vi "[ex ce] Curve Length.vi"() -> ()   [LabVIEW 2021]
doc: "CE-Math example.\n\n::: CalcExpress Toolkit :::\nCopyright (c) 2000-2026 Konstantin Shifershteyn. All rights reserved."
uses:
  ce exmpl - 1D difference info.ctl
  <vilib>/gmath/NI_Gmath.lvlib
panel:
  out "max relative difference":T1={"index"=-1, "absolute difference"=0.0, "relative difference, %"=0.0} {"relative difference, %" format="%#.6g"; "absolute difference" format="%#.6g"}
  out "max absolute difference":T1={"index"=-1, "absolute difference"=0.0, "relative difference, %"=0.0} {"relative difference, %" format="%#.6g"; "absolute difference" format="%#.6g"}
  in  "formula info":cluster{"formula":string, "x-variable":string}={"formula"="sinc(x)+sin(2*x)+sin(3*x)+sin(2*x*x)", "x-variable"="x"}
  in  "end":dbl=4.0 format="%.2f"
  in  "start":dbl format="%.2f"
  out "speed ratio":dbl format="%.3f"
  out "GM ticks":u32 caption="ms"
  out "CE ticks":u32 caption="ms"
  out "CE Graph":cluster{"x":dbl[], "f(x)":dbl[]}[](graph) caption="CalcExpress"
  out "GM Graph":cluster{"x":dbl[], "f(x)":dbl[]}[](graph) caption="G Math"
  # "NOTE    CalcExpress uses (^) operator to perform bitwise-XOR operation but not exponentiation operation.\nYou have to use double-asterisk (**) operator to compute an exponent in a CalcExpress expression. For sample, x**y ."
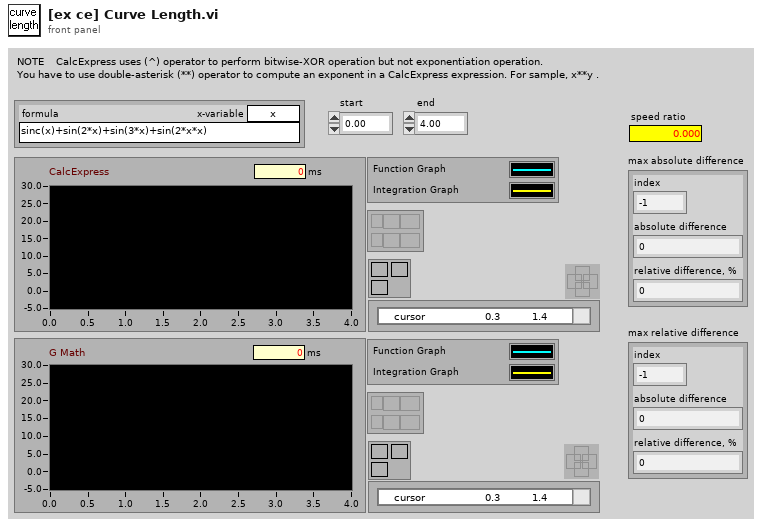
[diagram p1: front panel]
types:
  T1 = typedef "ce exmpl - 1D difference info.ctl" = cluster{"index":i32, "absolute difference":dbl, "relative difference, %":dbl}
  T2 = cluster{"X Values":dbl[], "Curve Length":dbl[]}[]
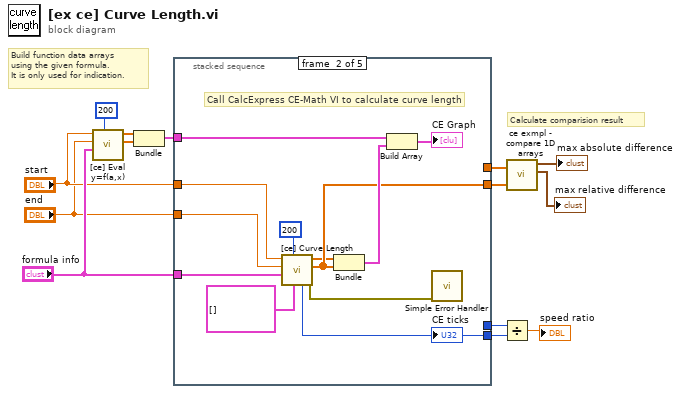
[diagram p0: block diagram]
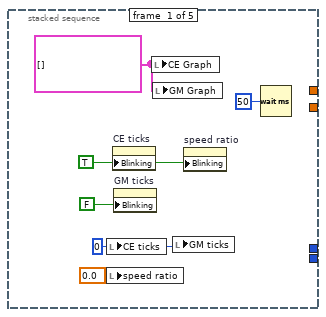
[diagram p2: hidden frame]
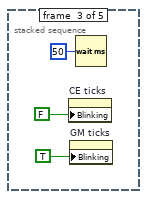
[diagram p3: hidden frame]
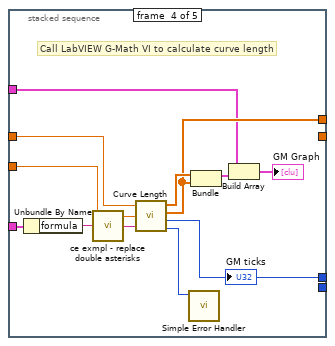
[diagram p4: hidden frame]
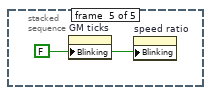
[diagram p5: hidden frame]
diagram:
  # "Calculate comparision result"
  # "Build function data arrays\nusing the given formula.\nIt is only used for indication."
  n1 = call "[ce] Eval y=f(a,x).vi"("# points"=u32 200, "formula info"="formula info", "end"="end", "start"="start") -> ("Y Values"=w6:dbl[], "X Values"=w7:dbl[])  [unwired: 4 in, 2 out]
  n2 = Bundle("X Values"=w7, "Y Values"=w6) -> (w5:cluster{"X Values":dbl[], "Y Values":dbl[]})  [unwired: 1 in]
  n3 = stacked-sequence {
    tunnel: "start" -> [_ w24 _ w43 _]
    tunnel: "end" -> [_ w23 _ w44 _]
    tunnel: "formula info" -> [_ w25 _ w42 _]
    tunnel: [_ w31 _ _ _] -> w14
    tunnel: [_ _ _ w45 _] -> w12
    tunnel: [_ _ _ w37 _] -> w11
    tunnel: [_ w28 _ _ _] -> w10
    tunnel: w5 -> [_ w21 _ w36 _]
    frame #0 {
      w15 = cluster{"x":dbl[], "f(x)":dbl[]}[] [] ("CE Graph")
      w17 = u32 0 ("CE ticks")
      w19 = TRUE ("Write Attribute")
      n4 = local write "CE ticks"(w17) -> ()
      n5 = local write "speed ratio"(0.0 ("speed ratio")) -> ()
      n6 = property on="CE ticks" class="DigNum (strict)"("Blinking"=w19) -> ()  [unwired: 2 in, 2 out]
      n7 = property on="GM ticks" class="DigNum (strict)"("Blinking"=FALSE ("Write Attribute")) -> ()  [unwired: 2 in, 2 out]
      n8 = local write "CE Graph"(w15) -> ()
      n9 = local write "GM Graph"(w15) -> ()
      n10 = local write "GM ticks"(w17) -> ()
      n11 = property on="speed ratio" class="DigNum (strict)"("Blinking"=w19) -> ()  [unwired: 2 in, 2 out]
      n12 = Wait (ms)(milliseconds to wait=u32 50) -> ()  [unwired: 1 out]
    }
    frame #1 {
      # "Call CalcExpress CE-Math VI to calculate curve length"
      n13 = call "[ce] Curve Length.vi"("parameters"=cluster{"name":string, "value":dbl}[] [] ("additional parameters"), "# points"=u32 200, "formula info"=w25, "end"=w23, "start"=w24) -> ("error out"=w32:errorcluster, "ticks"=w31:u32, "Curve Length"=w28:dbl[], "X Values"=w27:dbl[])  [unwired: 3 in]
      "CE ticks" <- w31
      n14 = Bundle("X Values"=w27, "Curve Length"=w28) -> (w30:cluster{"X Values":dbl[], "Curve Length":dbl[]})  [unwired: 1 in]
      n15 = Build Array(w21, w30) -> (→"CE Graph":T2)
      n16 = call <vilib>:"Simple Error Handler.vi"("error in (no error)"=w32) -> ()  [unwired: 4 in, 5 out]
    }
    frame #2 {
      n17 = property on="CE ticks" class="DigNum (strict)"("Blinking"=FALSE ("Write Attribute")) -> ()  [unwired: 2 in, 2 out]
      n18 = property on="GM ticks" class="DigNum (strict)"("Blinking"=TRUE ("Write Attribute")) -> ()  [unwired: 2 in, 2 out]
      n19 = Wait (ms)(milliseconds to wait=u32 50) -> ()  [unwired: 1 out]
    }
    frame #3 {
      # "Call LabVIEW G-Math VI to calculate curve length"
      n20 = Unbundle By Name(w42) -> ("formula"=w41:string)
      n21 = call "ce exmpl - replace double asterisks .vi"() -> ()  [unwired: 5 in, 1 out]
      n22 = call <vilib>:"Curve Length.vi"("start"=w43, "end"=w44, "formula"=w41) -> ("X Values"=w39:dbl[], "Curve Length"=w37:dbl[], "ticks"=w45:u32, "error"=w46:i32)
      "GM ticks" <- w45
      n23 = call <vilib>:"Simple Error Handler.vi"("error code (no error:0)"=w46) -> ()  [unwired: 4 in, 5 out]
      n24 = Bundle("X Values"=w39, "Curve Length"=w37) -> (w38:cluster{"X Values":dbl[], "Curve Length":dbl[]})  [unwired: 1 in]
      n25 = Build Array(w36, w38) -> (→"GM Graph":T2)
    }
    frame #4 {
      w47 = FALSE ("Write Attribute")
      n26 = property on="GM ticks" class="DigNum (strict)"("Blinking"=w47) -> ()  [unwired: 2 in, 2 out]
      n27 = property on="speed ratio" class="DigNum (strict)"("Blinking"=w47) -> ()  [unwired: 2 in, 2 out]
    }
  }
  n28 = Divide(x=w12, y=w14) -> (x/y=→"speed ratio":dbl)
  n29 = call "ce exmpl - compare 1D arrays.vi"("checking array B"=w10, "standard array A"=w11) -> ("max relative difference"=→"max relative difference":T1, "max absolute difference"=→"max absolute difference":T1)  [unwired: 1 in, 2 out]
